vi "Import Bitfile Scalars.vi"   [LabVIEW 2020, in "Scripting API.lvlib"]
doc: "Handles typical import operations, for the control and indicator registers contained in the bitfile configured for the target FPGA addon custom device."
uses:
  Scripting API.lvlib
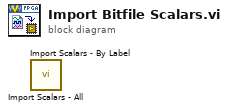
[diagram p0: block diagram]
diagram:
  n1 = call "Import Scalars - All.vi"() -> ()  [unwired: 9 in, 3 out]
  n2 = call "Import Scalars - By Label.vi"() -> ()  [unwired: 9 in, 3 out]
